vi "Load Client.vi"(6 "Code":string="28588716A182460064", 8 "error in":errorcluster, 9 "Data":i32, 10 "Mode":T3(ring), 11 "Station":string(combo)="Load") -> (0 "error out":errorcluster, 1 "string":T2, 2 "test state":T1, 3 "Comm ok?":bool)   [LabVIEW 2012]
uses:
  read_Array.vi
  write_Num.vi
  write_String.vi
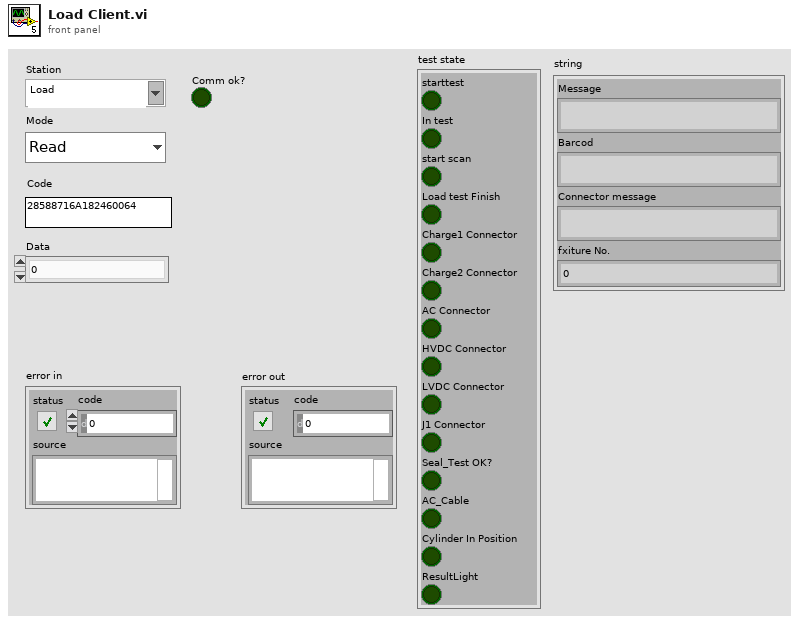
[diagram p1: front panel]
types:
  T1 = cluster{"starttest":bool, "In test":bool, "start scan":bool, "Load test Finish":bool, "Charge1 Connector":bool, "Charge2 Connector":bool, "AC Connector":bool, "HVDC Connector":bool, "LVDC Connector":bool, "J1 Connector":bool, "Seal_Test OK?":bool, "AC_Cable":bool, "Cylinder In Position":bool, "ResultLight":bool}
  T2 = cluster{"Message":string, "Barcod":string, "Connector message":string, "fxiture No.":dbl}
  T3 = enum16{"Read", "Write Code", "Write Para", "Write FIS PASS", "Write FIS FAIL", "In Test", "Write Result PASS", "Write Result FAIL", "Leakage Start"}
  T4 = cluster{"starttest":bool, "In test":bool, "start scan":bool, "test Finish":bool, "Charge1 Connector":bool, "Charge2 Connector":bool, "AC Connector":bool, "HVDC Connector":bool, "LVDC Connector":bool, "J1 Connector":bool, "Seal_Test OK?":bool, "Wire Exist":bool, "Cylinder In Position":bool, "on going":bool}
  T5 = cluster{"Message":string, "Barcod":string, "Connector message":string, "Numeric":dbl}
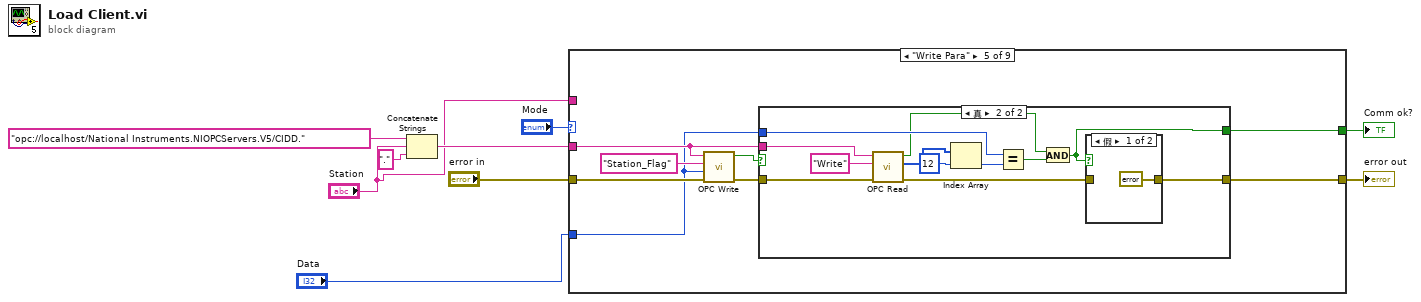
[diagram p0: block diagram]
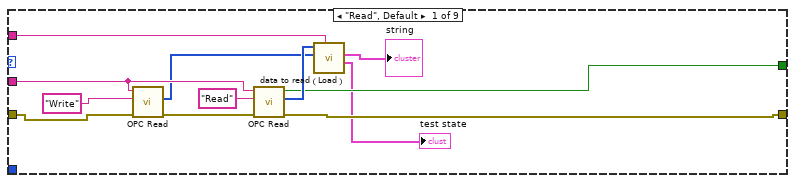
[diagram p2: hidden frame]
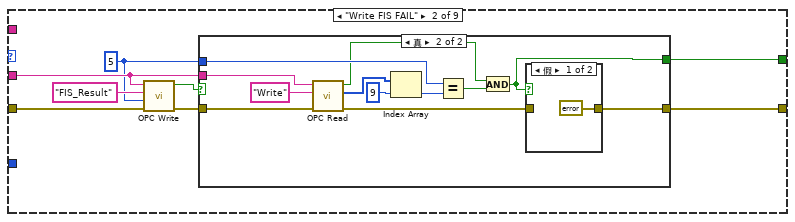
[diagram p3: hidden frame]
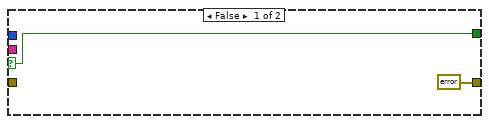
[diagram p4: hidden frame]
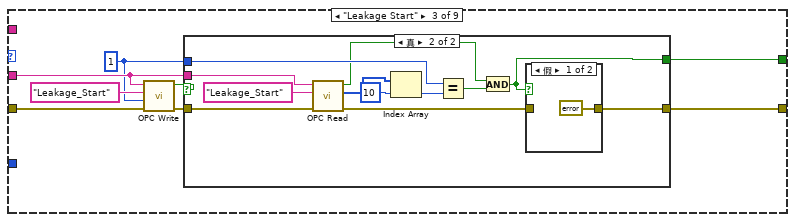
[diagram p6: hidden frame]
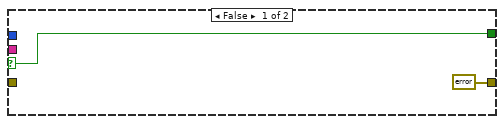
[diagram p7: hidden frame]
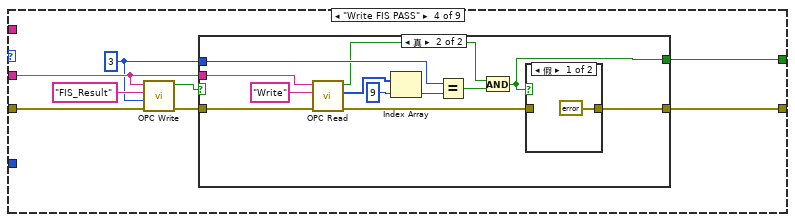
[diagram p9: hidden frame]
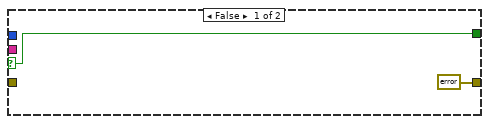
[diagram p10: hidden frame]
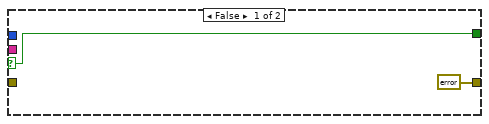
[diagram p12: hidden frame]
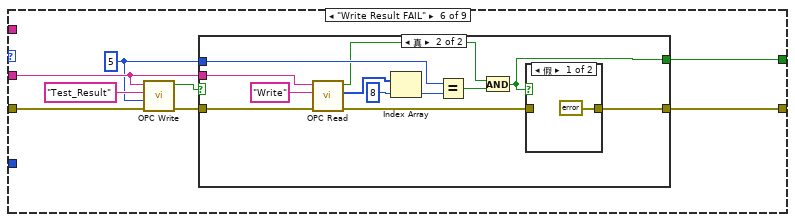
[diagram p14: hidden frame]
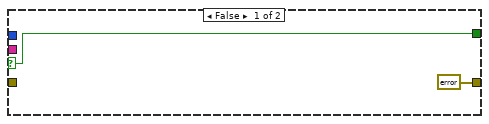
[diagram p15: hidden frame]
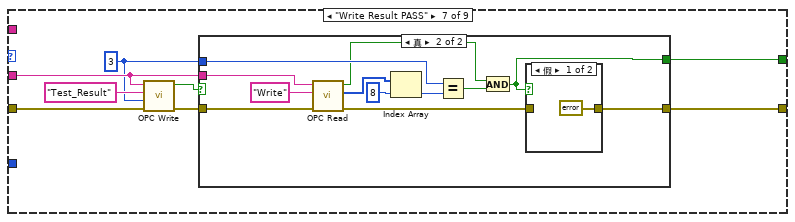
[diagram p17: hidden frame]
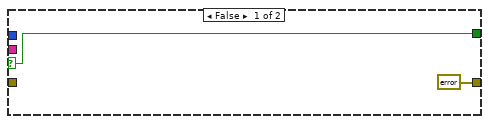
[diagram p18: hidden frame]
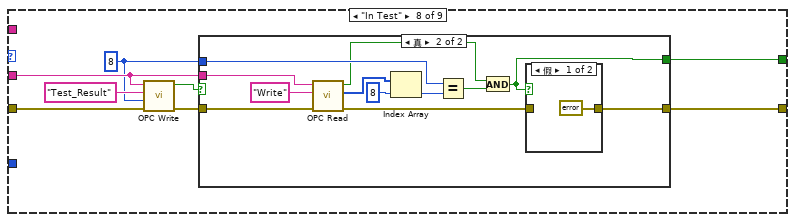
[diagram p20: hidden frame]
diagram:
  n1 = Concatenate Strings("opc://localhost/National Instruments.NIOPCServers.V5/CIDD." ("URL"), "Station", "." ("string")) -> (w7:string)
  n2 = case shown="\"Write Para\"" "Mode" {
    tunnel: w7 -> [w15 w27 w51 w75 w99 w121 w145 w169 w193]
    tunnel: [w20 w26 w50 w74 w98 w119 w143 w167 w191] -> w3
    tunnel: [w18 w25 w49 w73 w97 w120 w144 w168 w192] -> w5
    tunnel: "error in" -> [w12 w23 w47 w71 w95 w124 w148 w172 w196]
    tunnel: "Station" -> [w16 _ _ _ _ _ _ _ _]
    tunnel: "Data" -> [_ _ _ _ w94 _ _ _ _]
    frame "Read", Default {
      n3 = call-poly "OPC Read.vi"("错误输入（无错误）"=w12, "Address"="Write", "URL"=w15) -> ("error out"=w14:errorcluster, "Value"=w11:u8[])  [unwired: 6 in, 1 out]
      n4 = call-poly "OPC Read.vi"("错误输入（无错误）"=w14, "Address"="Read", "URL"=w15) -> ("error out"=w20:errorcluster, "Value"=w19:u8[], "ok?"=w18:bool)  [unwired: 6 in]
      n5 = call "data to read（Load）.vi"("Station"=w16, "Write data"=w11, "read data"=w19) -> ("test state"=→"test state":T4, "string"=→"string":T5)  [unwired: 7 in]
    }
    frame "Write FIS FAIL" {
      w22 = 5 ("Value")
      n6 = call-poly "OPC Write.vi"("错误输入（无错误）"=w23, "Value"=w22, "Address"="FIS_Result", "URL"=w27) -> ("error out"=w28:errorcluster, "ok?"=w24:bool)  [unwired: 6 in]
      n7 = case shown="真" w24 {
        selector: w24 -> [w30 _]
        tunnel: w28 -> [_ w42]
        tunnel: w27 -> [_ w41]
        tunnel: [errorcluster {"status"=FALSE, "code"=10001, "source"="Write Error"} ("error out") w33] -> w26
        tunnel: w22 -> [_ w37]
        tunnel: [w30 w34] -> w25
        frame False {
        }
        frame True {
          n8 = call-poly "OPC Read.vi"("错误输入（无错误）"=w42, "Address"="Write", "URL"=w41) -> ("error out"=w32:errorcluster, "Value"=w38:u8[], "ok?"=w35:bool)  [unwired: 6 in]
          n9 = Index Array(array=w38, index=9) -> (element=w40:u8)
          n10 = Equal?(x=w37, y=w40) -> (x = y?=w36:bool)
          n11 = And(x=w35, y=w36) -> (x .and. y?=w34:bool)
          n12 = case shown="假" w34 {
            tunnel: [errorcluster {"status"=FALSE, "code"=10001, "source"="Check Error"} ("error out") w45] -> w33
            tunnel: w32 -> [_ w45]
            frame False {
            }
            frame True {
            }
          }
        }
      }
    }
    frame "Leakage Start" {
      w46 = 1 ("Value")
      n13 = call-poly "OPC Write.vi"("错误输入（无错误）"=w47, "Value"=w46, "Address"="Leakage_Start", "URL"=w51) -> ("error out"=w52:errorcluster, "ok?"=w48:bool)  [unwired: 6 in]
      n14 = case shown="真" w48 {
        selector: w48 -> [w54 _]
        tunnel: w52 -> [_ w66]
        tunnel: w51 -> [_ w65]
        tunnel: [errorcluster {"status"=FALSE, "code"=10001, "source"="Write Error"} ("error out") w57] -> w50
        tunnel: w46 -> [_ w61]
        tunnel: [w54 w58] -> w49
        frame False {
        }
        frame True {
          n15 = call-poly "OPC Read.vi"("错误输入（无错误）"=w66, "Address"="Leakage_Start", "URL"=w65) -> ("error out"=w56:errorcluster, "Value"=w62:u8[], "ok?"=w59:bool)  [unwired: 6 in]
          n16 = Index Array(array=w62, index=10) -> (element=w64:u8)
          n17 = Equal?(x=w61, y=w64) -> (x = y?=w60:bool)
          n18 = And(x=w59, y=w60) -> (x .and. y?=w58:bool)
          n19 = case shown="假" w58 {
            tunnel: [errorcluster {"status"=FALSE, "code"=10001, "source"="Check Error"} ("error out") w69] -> w57
            tunnel: w56 -> [_ w69]
            frame False {
            }
            frame True {
            }
          }
        }
      }
    }
    frame "Write FIS PASS" {
      w70 = 3 ("Value")
      n20 = call-poly "OPC Write.vi"("错误输入（无错误）"=w71, "Value"=w70, "Address"="FIS_Result", "URL"=w75) -> ("error out"=w76:errorcluster, "ok?"=w72:bool)  [unwired: 6 in]
      n21 = case shown="真" w72 {
        selector: w72 -> [w78 _]
        tunnel: w76 -> [_ w90]
        tunnel: w75 -> [_ w89]
        tunnel: [errorcluster {"status"=FALSE, "code"=10001, "source"="Write Error"} ("error out") w81] -> w74
        tunnel: w70 -> [_ w85]
        tunnel: [w78 w82] -> w73
        frame False {
        }
        frame True {
          n22 = call-poly "OPC Read.vi"("错误输入（无错误）"=w90, "Address"="Write", "URL"=w89) -> ("error out"=w80:errorcluster, "Value"=w86:u8[], "ok?"=w83:bool)  [unwired: 6 in]
          n23 = Index Array(array=w86, index=9) -> (element=w88:u8)
          n24 = Equal?(x=w85, y=w88) -> (x = y?=w84:bool)
          n25 = And(x=w83, y=w84) -> (x .and. y?=w82:bool)
          n26 = case shown="假" w82 {
            tunnel: [errorcluster {"status"=FALSE, "code"=10001, "source"="Check Error"} ("error out") w93] -> w81
            tunnel: w80 -> [_ w93]
            frame False {
            }
            frame True {
            }
          }
        }
      }
    }
    frame "Write Para" {
      n27 = call-poly "OPC Write.vi"("错误输入（无错误）"=w95, "Value"=w94, "Address"="Station_Flag", "URL"=w99) -> ("error out"=w100:errorcluster, "ok?"=w96:bool)  [unwired: 6 in]
      n28 = case shown="真" w96 {
        selector: w96 -> [w102 _]
        tunnel: w100 -> [_ w114]
        tunnel: w99 -> [_ w113]
        tunnel: [errorcluster {"status"=FALSE, "code"=10001, "source"="Write Error"} ("error out") w105] -> w98
        tunnel: w94 -> [_ w109]
        tunnel: [w102 w106] -> w97
        frame False {
        }
        frame True {
          n29 = call-poly "OPC Read.vi"("错误输入（无错误）"=w114, "Address"="Write", "URL"=w113) -> ("error out"=w104:errorcluster, "Value"=w110:u8[], "ok?"=w107:bool)  [unwired: 6 in]
          n30 = Index Array(array=w110, index=12) -> (element=w112:u8)
          n31 = Equal?(x=w109, y=w112) -> (x = y?=w108:bool)
          n32 = And(x=w107, y=w108) -> (x .and. y?=w106:bool)
          n33 = case shown="假" w106 {
            tunnel: [errorcluster {"status"=FALSE, "code"=10001, "source"="Check Error"} ("error out") w117] -> w105
            tunnel: w104 -> [_ w117]
            frame False {
            }
            frame True {
            }
          }
        }
      }
    }
    frame "Write Result FAIL" {
      w118 = 5 ("Value")
      n34 = call-poly "OPC Write.vi"("错误输入（无错误）"=w124, "Value"=w118, "Address"="Test_Result", "URL"=w121) -> ("error out"=w122:errorcluster, "ok?"=w123:bool)  [unwired: 6 in]
      n35 = case shown="真" w123 {
        selector: w123 -> [w126 _]
        tunnel: w122 -> [_ w138]
        tunnel: w121 -> [_ w137]
        tunnel: [errorcluster {"status"=FALSE, "code"=10001, "source"="Write Error"} ("error out") w129] -> w119
        tunnel: w118 -> [_ w133]
        tunnel: [w126 w130] -> w120
        frame False {
        }
        frame True {
          n36 = call-poly "OPC Read.vi"("错误输入（无错误）"=w138, "Address"="Write", "URL"=w137) -> ("error out"=w128:errorcluster, "Value"=w134:u8[], "ok?"=w131:bool)  [unwired: 6 in]
          n37 = Index Array(array=w134, index=8) -> (element=w136:u8)
          n38 = Equal?(x=w133, y=w136) -> (x = y?=w132:bool)
          n39 = And(x=w131, y=w132) -> (x .and. y?=w130:bool)
          n40 = case shown="假" w130 {
            tunnel: [errorcluster {"status"=FALSE, "code"=10001, "source"="Check Error"} ("error out") w141] -> w129
            tunnel: w128 -> [_ w141]
            frame False {
            }
            frame True {
            }
          }
        }
      }
    }
    frame "Write Result PASS" {
      w142 = 3 ("Value")
      n41 = call-poly "OPC Write.vi"("错误输入（无错误）"=w148, "Value"=w142, "Address"="Test_Result", "URL"=w145) -> ("error out"=w146:errorcluster, "ok?"=w147:bool)  [unwired: 6 in]
      n42 = case shown="真" w147 {
        selector: w147 -> [w150 _]
        tunnel: w146 -> [_ w162]
        tunnel: w145 -> [_ w161]
        tunnel: [errorcluster {"status"=FALSE, "code"=10001, "source"="Write Error"} ("error out") w153] -> w143
        tunnel: w142 -> [_ w157]
        tunnel: [w150 w154] -> w144
        frame False {
        }
        frame True {
          n43 = call-poly "OPC Read.vi"("错误输入（无错误）"=w162, "Address"="Write", "URL"=w161) -> ("error out"=w152:errorcluster, "Value"=w158:u8[], "ok?"=w155:bool)  [unwired: 6 in]
          n44 = Index Array(array=w158, index=8) -> (element=w160:u8)
          n45 = Equal?(x=w157, y=w160) -> (x = y?=w156:bool)
          n46 = And(x=w155, y=w156) -> (x .and. y?=w154:bool)
          n47 = case shown="假" w154 {
            tunnel: [errorcluster {"status"=FALSE, "code"=10001, "source"="Check Error"} ("error out") w165] -> w153
            tunnel: w152 -> [_ w165]
            frame False {
            }
            frame True {
            }
          }
        }
      }
    }
    frame "In Test" {
      w166 = 8 ("Value")
      n48 = call-poly "OPC Write.vi"("错误输入（无错误）"=w172, "Value"=w166, "Address"="Test_Result", "URL"=w169) -> ("error out"=w170:errorcluster, "ok?"=w171:bool)  [unwired: 6 in]
      n49 = case shown="真" w171 {
        selector: w171 -> [w174 _]
        tunnel: w170 -> [_ w186]
        tunnel: w169 -> [_ w185]
        tunnel: [errorcluster {"status"=FALSE, "code"=10001, "source"="Write Error"} ("error out") w177] -> w167
        tunnel: w166 -> [_ w181]
        tunnel: [w174 w178] -> w168
        frame False {
        }
        frame True {
          n50 = call-poly "OPC Read.vi"("错误输入（无错误）"=w186, "Address"="Write", "URL"=w185) -> ("error out"=w176:errorcluster, "Value"=w182:u8[], "ok?"=w179:bool)  [unwired: 6 in]
          n51 = Index Array(array=w182, index=8) -> (element=w184:u8)
          n52 = Equal?(x=w181, y=w184) -> (x = y?=w180:bool)
          n53 = And(x=w179, y=w180) -> (x .and. y?=w178:bool)
          n54 = case shown="假" w178 {
            tunnel: [errorcluster {"status"=FALSE, "code"=10001, "source"="Check Error"} ("error out") w189] -> w177
            tunnel: w176 -> [_ w189]
            frame False {
            }
            frame True {
            }
          }
        }
      }
    }
    frame "Write Code" {
      n55 = call-poly "OPC Write.vi"("错误输入（无错误）"=w196, "Value"="Code", "Address"="Scan_Barcode", "URL"=w193) -> ("error out"=w194:errorcluster, "ok?"=w195:bool)  [unwired: 6 in]
      n56 = case shown="真" w195 {
        selector: w195 -> [w198 _]
        tunnel: w194 -> [_ w214]
        tunnel: w193 -> [_ w213]
        tunnel: [errorcluster {"status"=FALSE, "code"=10001, "source"="Write Error"} ("error out") w207] -> w191
        tunnel: "Code" -> [_ w211]
        tunnel: [w198 w208] -> w192
        frame False {
        }
        frame True {
          w204 = 31 ("index")
          n57 = call-poly "OPC Read.vi"("错误输入（无错误）"=w214, "Address"="Write", "URL"=w213) -> ("error out"=w206:errorcluster, "Value"=w205:u8[], "ok?"=w209:bool)  [unwired: 6 in]
          n58 = Increment(x=w204) -> (x+1=w203:i32)
          n59 = Index Array(array=w205, index #1=30 ("index"), index #2=w204) -> (element #2=w202:u8)  [unwired: 1 out]
          n60 = Array Subset(array=w205, index=w203, length=w202) -> (w201:u8[])
          n61 = Byte Array To String(unsigned byte array=w201) -> (string=w200:string)
          n62 = Equal?(x=w211, y=w200) -> (x = y?=w210:bool)
          n63 = And(x=w209, y=w210) -> (x .and. y?=w208:bool)
          n64 = case shown="真" w208 {
            tunnel: [errorcluster {"status"=FALSE, "code"=10001, "source"="Check Error"} ("error out") w217] -> w207
            tunnel: w206 -> [_ w217]
            frame False {
            }
            frame True {
            }
          }
        }
      }
    }
  }
  "Comm ok?" <- w5
  "error out" <- w3
